vi "DialogCreateClass_HandleTemplatesDialog.vi"(8 "error in (no error)":errorcluster, 10 "AllTemplatesForThisProvider/InheritanceType(Base/Sub)":T1[](array[typedef]), 11 "ClassWriter in":refnum<class "ClassWriter.lvclass">) -> (0 "error out":errorcluster, 2 "TemplatesOut":T1[](array[typedef]), 3 "RefreshClassTemplates":bool)   [LabVIEW 2020, in "ClassWriterNative.lvclass"]
uses:
  <resource>/Framework/Providers/Open_GDS/ClassProviders/Provider_LvNativeClass/ClassWriterNative_class/ClassWriterNative.lvclass
  <resource>/Framework/Providers/Open_GDS/ClassProviders/Provider_BaseClassInterface/ClassTemplateType.ctl
  <resource>/Framework/Providers/Open_GDS/ClassProviders/Provider_BaseClassInterface/ClassWriter_class/ClassWriter.lvclass
  <vilib>/Utility/config.llb/Write Key (String).vi
  <resource>/Framework/Providers/Open_GDS/ClassProviders/Provider_LvNativeClass/ClassWriterNative_class/ClassWriterNative.lvclass/ClassWriterNative.ctl
  <vilib>/Utility/config.llb/NI_LVConfig.lvlib
panel:
  in  "RemoveTemplate":bool
  in  "AddTemplate":bool
  in  "Cancel":bool
  in  "Save":bool
  in  "Down":bool
  in  "Up":bool
  in  "ClassTemplates":i32(listbox) caption="Class Templates"
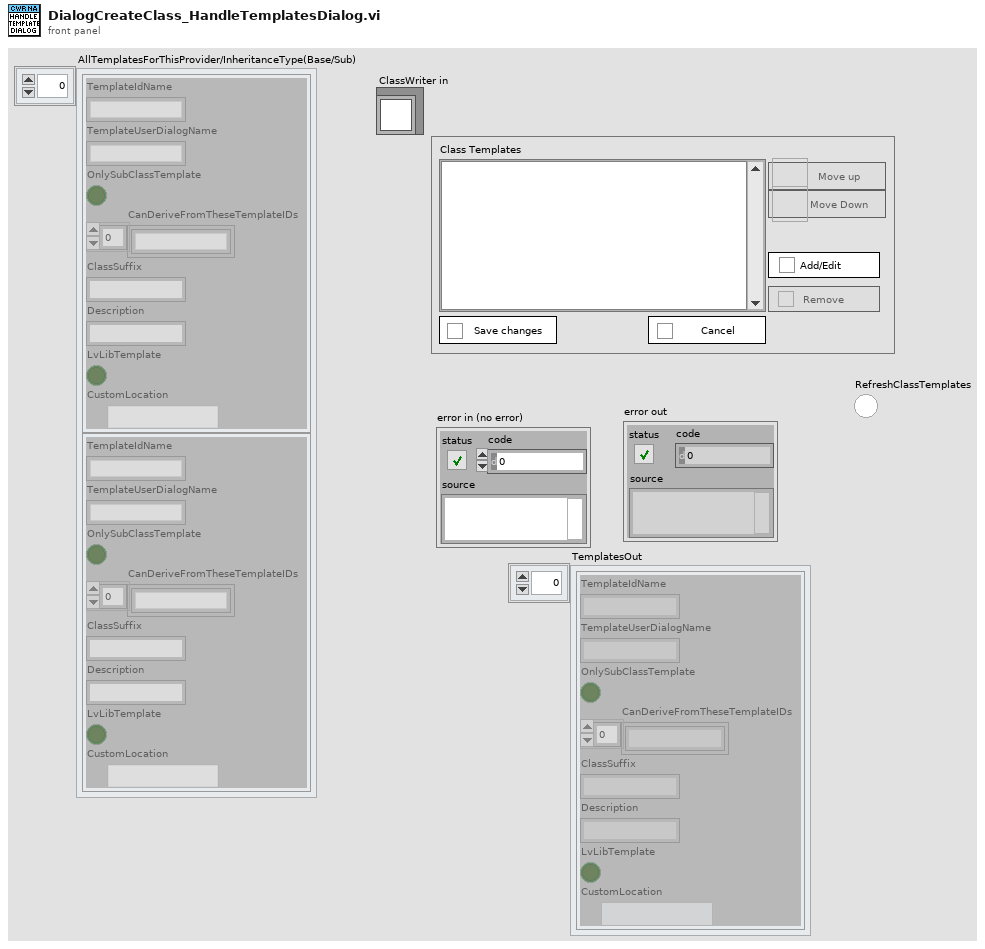
[diagram p1: front panel]
types:
  T1 = typedef "ClassWriter.lvclass/ClassTemplateType.ctl" = cluster{"TemplateIdName":string, "TemplateUserDialogName":string, "OnlySubClassTemplate":bool, "CanDeriveFromTheseTemplateIDs":string[], "ClassSuffix":string, "Description":string, "LvLibTemplate":bool, "CustomLocation":path}
  T2 = cluster{"Section":string, "TemplateIndexSelected":i32, "Templates":T1[], "RefreshClassTemplates":bool, "ProviderShortName":string, "TemplateFilter":cluster{"TemplateNamesSortOrder":string[], "HiddenTemplateNames":string[]}}
  T3 = enum8{"Enabled", "Disabled", "Disabled and Grayed Out"}
  T4 = cluster{"TemplateNamesSortOrder":string[], "HiddenTemplateNames":string[]}
  T5 = cluster{u32, "TemplateUserDialogName":string, bool}
  T6 = cluster{u32, "TemplateUserDialogName":string, bool}[]
  T7 = typedef "LVPoint32TypeDef.ctl" = cluster{"Horizontal":i32, "Vertical":i32}
  T8 = typedef "NI_LVConfig.lvlib/Config Data RefNum.ctl" = refnum<k1>
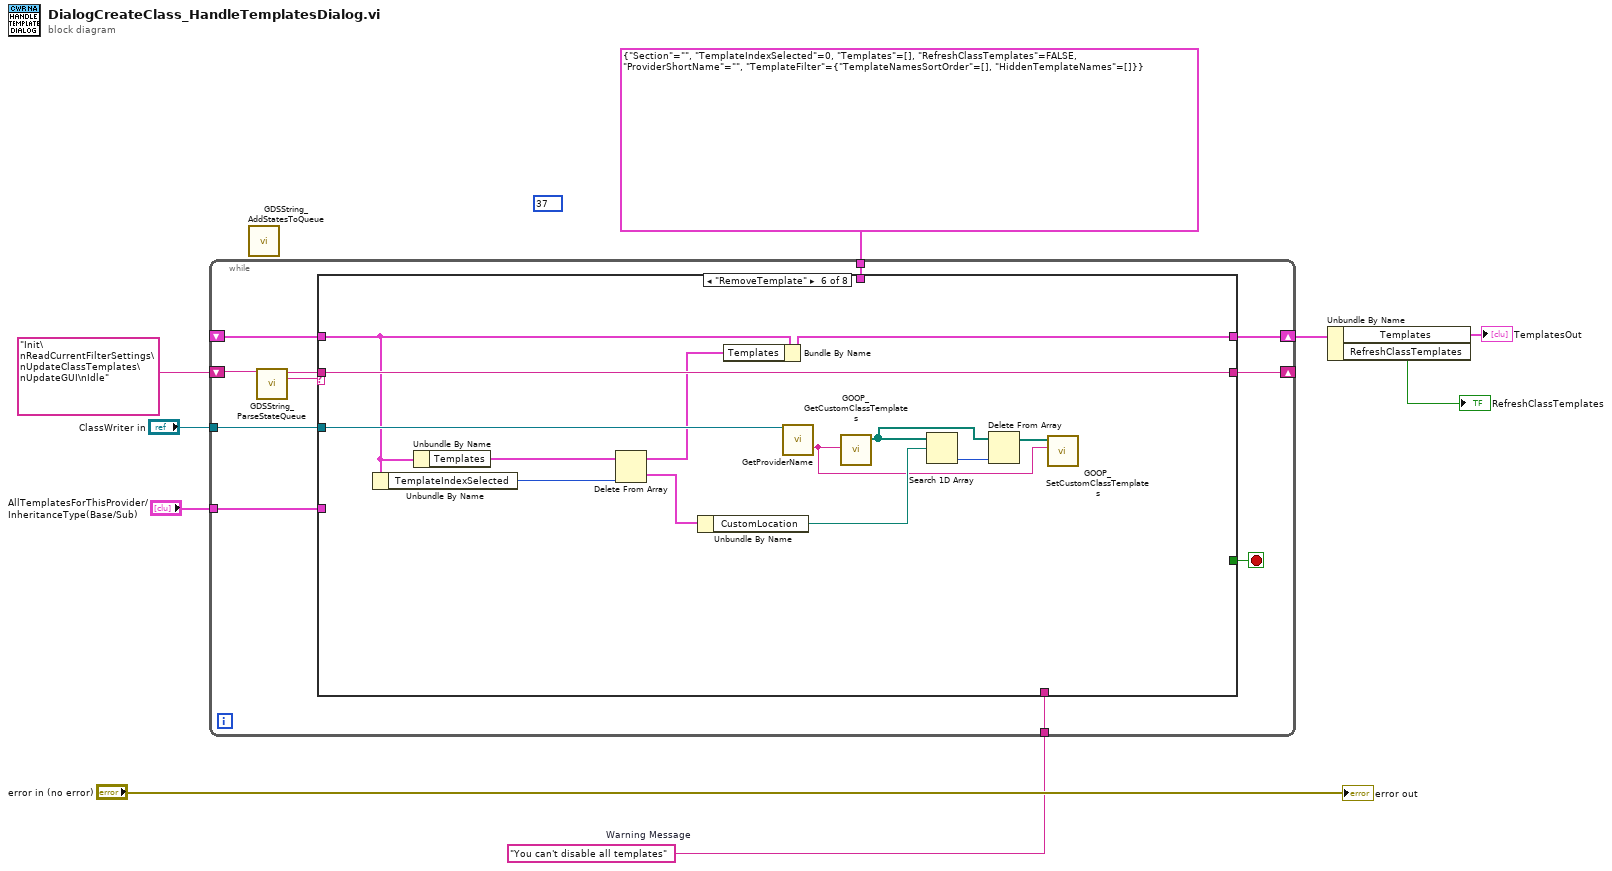
[diagram p0: block diagram]
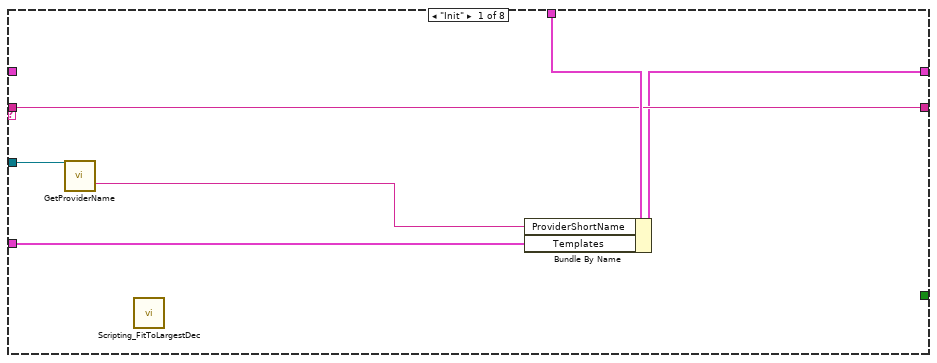
[diagram p2: hidden frame]
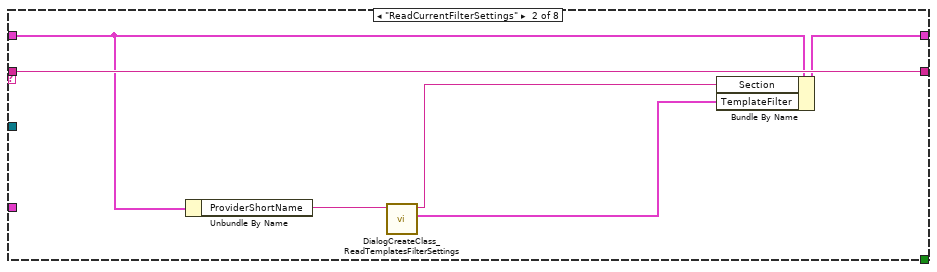
[diagram p3: hidden frame]
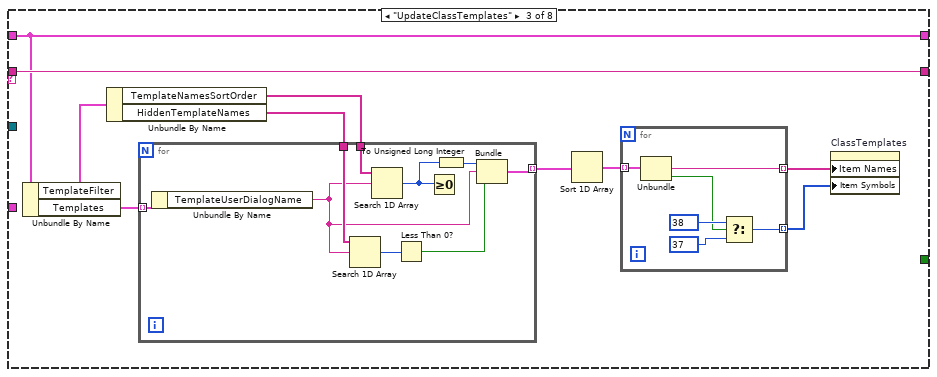
[diagram p4: hidden frame]
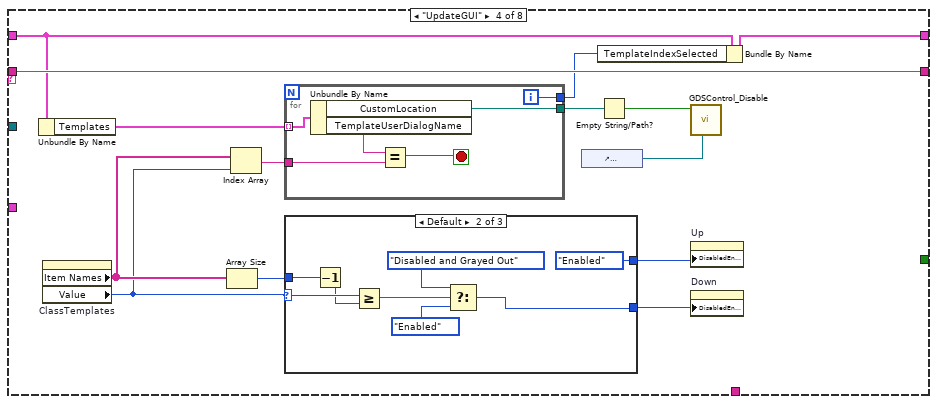
[diagram p5: hidden frame]
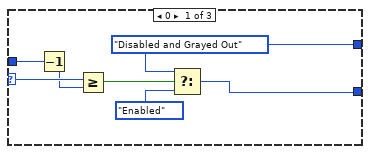
[diagram p6: hidden frame]
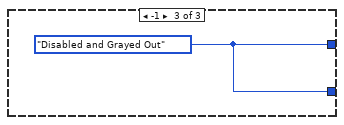
[diagram p7: hidden frame]
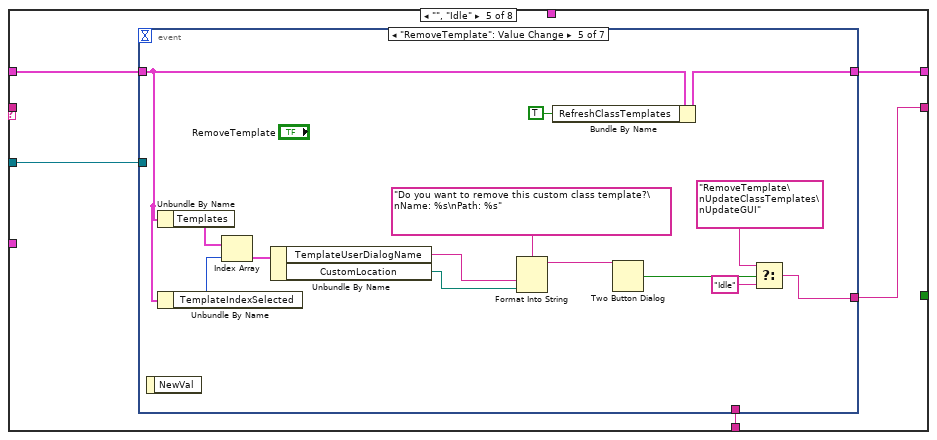
[diagram p8: hidden frame]
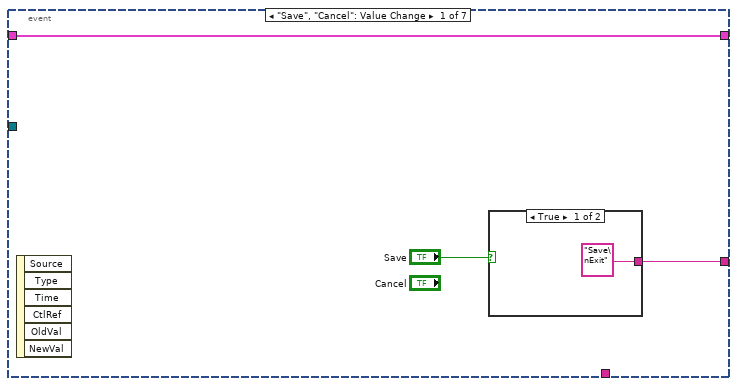
[diagram p9: hidden frame]
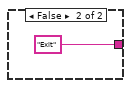
[diagram p10: hidden frame]
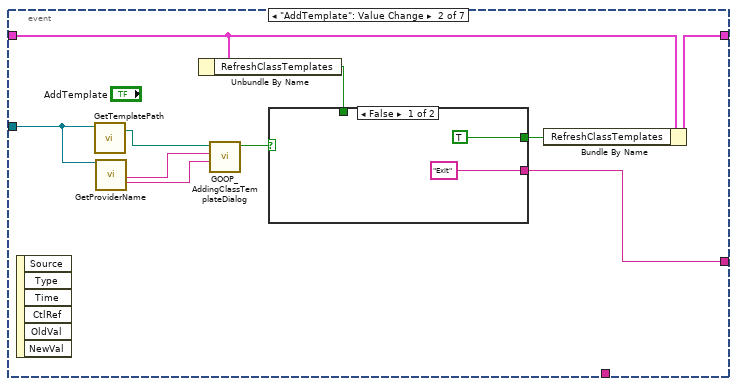
[diagram p11: hidden frame]
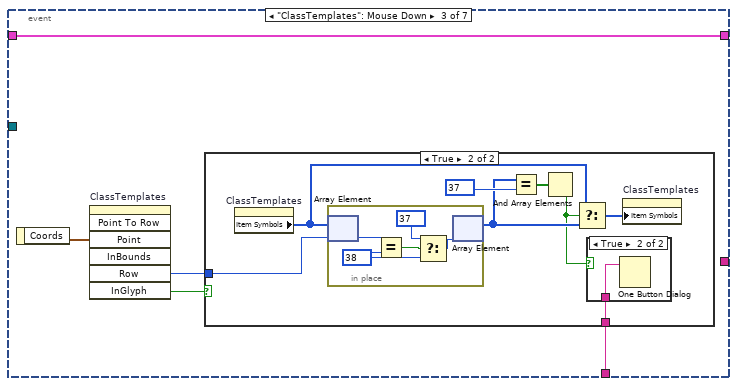
[diagram p13: hidden frame]
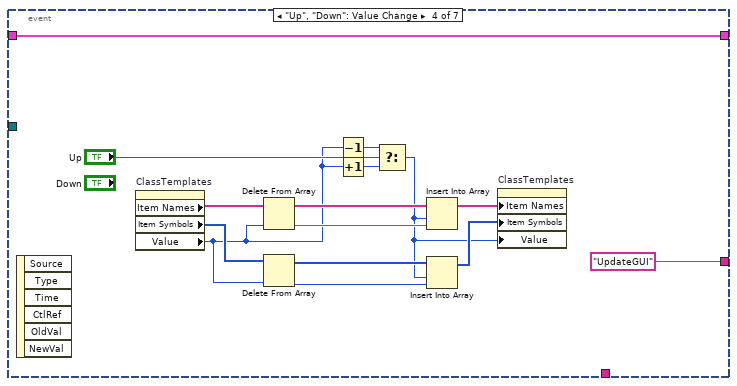
[diagram p16: hidden frame]
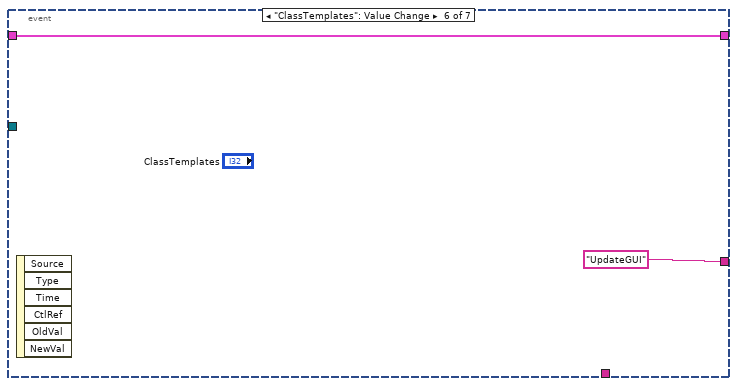
[diagram p17: hidden frame]
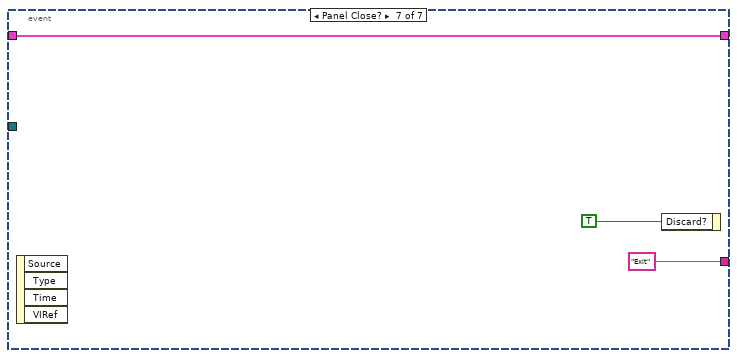
[diagram p18: hidden frame]
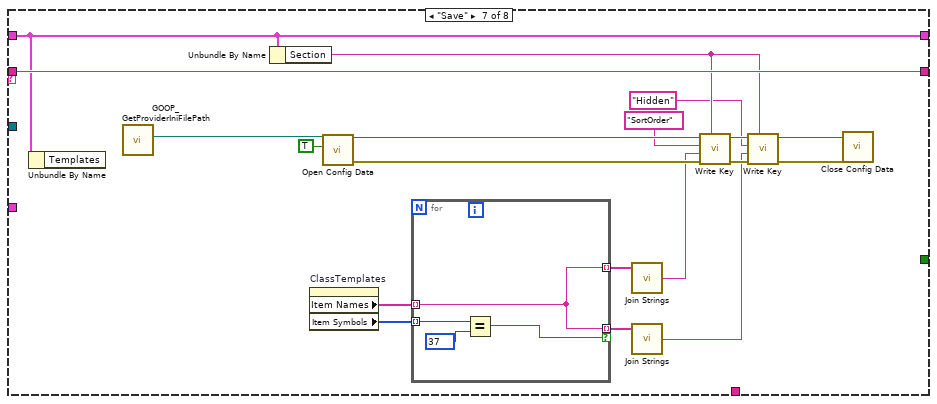
[diagram p19: hidden frame]
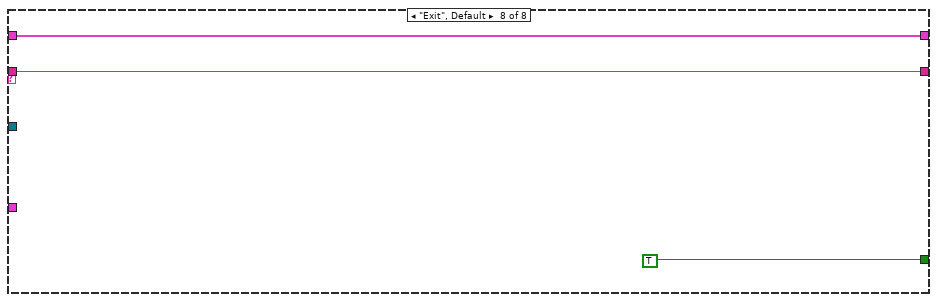
[diagram p20: hidden frame]
diagram:
  (unwired) 37
  w6 = "You can't disable all templates"  # Warning Message
  n1 = while {
    shift-right: [w18] -> _
    shift-left: "Init\nReadCurrentFilterSettings\nUpdateClassTemplates\nUpdateGUI\nIdle" ("Remaining States") -> [w19]
    tunnel: "AllTemplatesForThisProvider/InheritanceType(Base/Sub)" -> [w15]
    tunnel: T2 {"Section"="", "TemplateIndexSelected"=0, "Templates"=[], "RefreshClassTemplates"=FALSE, "ProviderShortName"="", "TemplateFilter"={"TemplateNamesSortOrder"=[], "HiddenTemplateNames"=[]}} -> [w14]
    shift-right: [w13] -> w3
    shift-left: _ -> [w12]
    tunnel: w6 -> [w11]
    tunnel: "ClassWriter in" -> [w10]
    stop <- w20 stop-if-true
    n2 = call <resource>:"GDSString_ParseStateQueue.vi"("State Queue"=w19) -> ("Remaining States"=w16:string, "Current State"=w17:string)  [unwired: 10 in, 3 out]
    n3 = case shown="\"RemoveTemplate\"" w17 {
      tunnel: [_ _ _ _ _ _ _ TRUE] -> w20
      tunnel: [w25 w32 w42 w71 w98 w182 w201 w207] -> w18
      tunnel: w16 -> [w25 w32 w42 w71 _ w182 w201 w207]
      tunnel: w15 -> [w23 _ _ _ _ _ _ _]
      tunnel: [w24 w30 w41 w61 w94 w172 w196 w206] -> w13
      tunnel: w14 -> [w26 _ _ _ _ _ _ _]
      tunnel: w12 -> [_ w28 w41 w59 w96 w176 w196 w206]
      tunnel: w11 -> [_ _ _ _ w97 _ _ _]
      tunnel: w10 -> [w22 _ _ _ w95 w181 _ _]
      frame "Init" {
        n4 = call-dynamic "GetProviderName.vi"("ClassWriter in"=w22) -> ("ShortName(Could be used in for INI Sections)"=w21:string)  [unwired: 14 in, 4 out]
        n5 = call <resource>:"Scripting_FitToLargestDec.vi"() -> ()  [unwired: 6 in, 2 out]
        n6 = Bundle By Name(cluster=w26, "ProviderShortName"=w21, "Templates"=w23) -> (w24:T2)
      }
      frame "ReadCurrentFilterSettings" {
        n7 = Unbundle By Name(w28) -> ("ProviderShortName"=w27:string)
        n8 = call <resource>:"DialogCreateClass_ReadTemplatesFilterSettings.vi"("ProviderShortName"=w27) -> ("TemplateFilter"=w31:T4, "Section"=w29:string)  [unwired: 9 in]
        n9 = Bundle By Name(cluster=w28, "Section"=w29, "TemplateFilter"=w31) -> (w30:T2)
      }
      frame "UpdateClassTemplates" {
        n10 = Unbundle By Name(w41) -> ("TemplateFilter"=w39:T4, "Templates"=w40:T1[])
        n11 = Unbundle By Name(w39) -> ("TemplateNamesSortOrder"=w38:string[], "HiddenTemplateNames"=w35:string[])
        n12 = for {
          tunnel: w40 -> [w57] mode=indexing
          tunnel: w38 -> [w56]
          tunnel: [w53] -> w37 mode=indexing
          tunnel: w35 -> [w52]
          n13 = Unbundle By Name(w57) -> ("TemplateUserDialogName"=w49:string)
          n14 = Search 1D Array(1D array=w52, element=w49) -> (index of element=w51:i32)  [unwired: 1 in]
          n15 = Search 1D Array(1D array=w56, element=w49) -> (index of element=w55:i32)  [unwired: 1 in]
          n16 = Less Than 0?(x=w51) -> (x < 0?=w50:bool)
          n17 = Greater Or Equal To 0?(x=w55) -> ()  [unwired: 1 out]
          n18 = To Unsigned Long Integer(number=w55) -> (unsigned 32bit integer=w54:u32)
          n19 = Bundle(w54, "TemplateUserDialogName"=w49, w50) -> (w53:T5)  [unwired: 1 in]
        }
        n20 = Sort 1D Array(array=w37) -> (sorted array=w36:T6)
        n21 = for {
          tunnel: w36 -> [w48] mode=indexing
          tunnel: [w45] -> w34 mode=indexing
          tunnel: [w44] -> w33 mode=indexing
          n22 = Unbundle(w48) -> ("TemplateUserDialogName"=w45:string, w43:bool)  [unwired: 1 out]
          n23 = Select(t=38, s=w43, f=37) -> (s? t:f=w44:i32)
        }
        n24 = property on="ClassTemplates" class="LstBox (strict)"("Item Names"=w34, "Item Symbols"=w33) -> ()  [unwired: 2 in, 2 out]
      }
      frame "UpdateGUI" {
        n25 = Unbundle By Name(w59) -> ("Templates"=w58:T1[])
        n26 = property on="ClassTemplates" class="LstBox (strict)"() -> ("Item Names"=w67:string[], "Value"=w66:i32)  [unwired: 2 in, 2 out]
        n27 = Array Size(array=w67) -> (size(s)=w68:i32)
        n28 = Index Array(array=w67, index=w66) -> (element=w65:string)
        n29 = for {
          tunnel: w58 -> [w77] mode=indexing
          tunnel: w65 -> [w75]
          tunnel: [w73] -> w64
          tunnel: [w72] -> w60
          i -> [w72]
          stop <- w74 stop-if-true
          n30 = Unbundle By Name(w77) -> ("CustomLocation"=w73:path, "TemplateUserDialogName"=w76:string)
          n31 = Equal?(x=w76, y=w75) -> (x = y?=w74:bool)
        }
        n32 = case shown="Default" w66 {
          selector: w66 -> [w84 w92 _]
          tunnel: [w79 T3."Enabled" ("Disabled") w93] -> w70
          tunnel: [w80 w88 w93] -> w69
          tunnel: w68 -> [w83 w91 _]
          frame 0 {
            w79 = T3."Disabled and Grayed Out" ("Disabled")
            n33 = Decrement(x=w83) -> (x-1=w82:i32)
            n34 = Greater Or Equal?(x=w84, y=w82) -> (x >= y?=w81:bool)
            n35 = Select(t=w79, s=w81, f=T3."Enabled" ("Disabled")) -> (s? t:f=w80:T3)
          }
          frame Default {
            n36 = Decrement(x=w91) -> (x-1=w90:i32)
            n37 = Greater Or Equal?(x=w92, y=w90) -> (x >= y?=w89:bool)
            n38 = Select(t=T3."Disabled and Grayed Out" ("Disabled"), s=w89, f=T3."Enabled" ("Disabled")) -> (s? t:f=w88:T3)
          }
          frame -1 {
            w93 = T3."Disabled and Grayed Out" ("Disabled")
          }
        }
        n39 = control-ref of="RemoveTemplate"() -> (w62:refnum<vi>)
        n40 = Bundle By Name(cluster=w59, "TemplateIndexSelected"=w60) -> (w61:T2)
        n41 = Empty String/Path?(string/path=w64) -> (empty?=w63:bool)
        n42 = call <resource>:"GDSControl_Disable.vi"("ControlRefnum(IgnoreIfNotWired)"=w62, "Disasble(True)"=w63) -> ()  [unwired: 9 in, 1 out]
        n43 = property on="Up" class="Bool"("DisabledEnum"=w70) -> ()  [unwired: 2 in, 2 out]
        n44 = property on="Down" class="Bool"("DisabledEnum"=w69) -> ()  [unwired: 2 in, 2 out]
      }
      frame "", "Idle" {
        n45 = event shown="[4] \"RemoveTemplate\": Value Change" {
          selector: _ -> [_ _ _ _ _ _ _]
          dyn-events: _ -> [_ _ _ _ _ _ _]
          timeout: _ -> [_ _ _ _ _ _ _]
          tunnel: [w101 w108 _ "UpdateGUI" w157 "UpdateGUI" "Exit"] -> w98
          tunnel: w97 -> [_ _ w118 _ _ _ _]
          tunnel: w96 -> [w99 w105 w117 w136 w152 w165 w167]
          tunnel: w95 -> [_ w113 _ _ _ _ _]
          tunnel: [w99 w107 w117 w136 w153 w165 w167] -> w94
          event "Save", "Cancel": Value Change {
            n46 = event-data() -> ()  [unwired: 1 in, 6 out]
            n47 = case shown="True" "Save" {
              tunnel: ["Save\nExit" "Exit"] -> w101
              frame True {
              }
              frame False {
              }
            }
          }
          event "AddTemplate": Value Change {
            n48 = event-data() -> ()  [unwired: 1 in, 6 out]
            n49 = call-dynamic "GetTemplatePath.vi"("ClassWriterIn"=w113) -> ("FolderPathOut"=w112:path)  [unwired: 14 in, 4 out]
            n50 = call-dynamic "GetProviderName.vi"("ClassWriter in"=w113) -> ("TranslatedProviderName"=w111:string, "ShortName(Could be used in for INI Sections)"=w110:string)  [unwired: 14 in, 3 out]
            n51 = Unbundle By Name(w105) -> ("RefreshClassTemplates"=w104:bool)
            n52 = call <resource>:"GOOP_AddingClassTemplateDialog.vi"("ShortName(Could be used in for INI Sections)"=w110, "TranslatedProviderName"=w111, "FolderPathOut"=w112) -> ("Cancelled"=w109:bool)  [unwired: 8 in]
            n53 = case shown="False" w109 {
              tunnel: ["Exit" _] -> w108
              tunnel: [TRUE w116] -> w106
              tunnel: w104 -> [_ w116]
              frame False {
              }
              frame True {
              }
            }
            n54 = Bundle By Name(cluster=w105, "RefreshClassTemplates"=w106) -> (w107:T2)
          }
          event "ClassTemplates": Mouse Down {
            n55 = event-data() -> ("Coords"=w121:T7)  [unwired: 1 in]
            n56 = invoke on="ClassTemplates" class="LstBox (strict)" method="Point To Row"("Point"=w121) -> ("Row"=w119:i32, "InGlyph"=w120:bool)  [unwired: 6 in, 5 out]
            n57 = case shown="True" w120 {
              tunnel: w119 -> [_ w129]
              tunnel: w118 -> [_ w122]
              frame False {
              }
              frame True {
                n58 = property on="ClassTemplates" class="LstBox (strict)"() -> ("Item Symbols"=w125:i32[])  [unwired: 2 in, 2 out]
                n59 = in-place {
                  w133 = 38
                  n60 = in-place-array #1(w125, w129) -> (w135:i32)
                  n61 = Equal?(x=w135, y=w133) -> (x = y?=w134:bool)
                  n62 = Select(t=37, s=w134, f=w133) -> (s? t:f=w131:i32)
                  n63 = in-place-array #1(w131) -> (w126:i32[])  [unwired: 1 out]
                }
                n64 = Equal?(x=w126, y=37) -> (x = y?=w127:bool[])
                n65 = And Array Elements(Boolean array=w127) -> (logical AND=w123:bool)
                n66 = Select(t=w125, s=w123, f=w126) -> (s? t:f=w124:i32[])
                n67 = case shown="True" w123 {
                  tunnel: w122 -> [_ w130]
                  frame False {
                  }
                  frame True {
                    n68 = One Button Dialog(message=w130) -> ()  [unwired: 1 in, 1 out]
                  }
                }
                n69 = property on="ClassTemplates" class="LstBox (strict)"("Item Symbols"=w124) -> ()  [unwired: 2 in, 2 out]
              }
            }
          }
          event "Up", "Down": Value Change {
            n70 = event-data() -> ()  [unwired: 1 in, 6 out]
            n71 = property on="ClassTemplates" class="LstBox (strict)"() -> ("Item Names"=w149:string[], "Item Symbols"=w148:i32[], "Value"=w139:i32)  [unwired: 2 in, 2 out]
            n72 = Delete From Array(array=w149, index=w139) -> (deleted portion=w145:string, array with subset deleted=w147:string[])  [unwired: 1 in]
            n73 = Delete From Array(array=w148, index=w139) -> (deleted portion=w144:i32, array with subset deleted=w146:i32[])  [unwired: 1 in]
            n74 = Decrement(x=w139) -> (x-1=w138:i32)
            n75 = Increment(x=w139) -> (x+1=w137:i32)
            n76 = Select(t=w138, s="Up", f=w137) -> (s? t:f=w140:i32)
            n77 = Insert Into Array(array=w147, index=w140, new element=w145) -> (w142:string[])
            n78 = Insert Into Array(array=w146, index=w140, new element=w144) -> (w141:i32[])
            n79 = property on="ClassTemplates" class="LstBox (strict)"("Item Names"=w142, "Item Symbols"=w141, "Value"=w140) -> ()  [unwired: 2 in, 2 out]
          }
          event "RemoveTemplate": Value Change {
            n80 = event-data() -> ()  [unwired: 1 in, 1 out]
            n81 = Unbundle By Name(w152) -> ("Templates"=w154:T1[])
            n82 = Unbundle By Name(w152) -> ("TemplateIndexSelected"=w163:i32)
            n83 = Index Array(array=w154, index=w163) -> (element=w162:T1)
            n84 = Unbundle By Name(w162) -> ("TemplateUserDialogName"=w161:string, "CustomLocation"=w160:path)
            n85 = Format Into String(format string="Do you want to remove this custom class template?\nName: %s\nPath: %s", w161, w160) -> (resulting string=w159:string)  [unwired: 2 in, 1 out]
            n86 = Bundle By Name(cluster=w152, "RefreshClassTemplates"=TRUE) -> (w153:T2)
            n87 = Two Button Dialog(message=w159) -> (T button?=w158:bool)  [unwired: 2 in]
            n88 = Select(t="RemoveTemplate\nUpdateClassTemplates\nUpdateGUI", s=w158, f="Idle") -> (s? t:f=w157:string)
          }
          event "ClassTemplates": Value Change {
            n89 = event-data() -> ()  [unwired: 1 in, 6 out]
          }
          event Panel Close? {
            n90 = event-data() -> ()  [unwired: 1 in, 4 out]
            n91 = event-data("Discard?"=TRUE) -> ()  [unwired: 1 in, 1 out]
          }
        }
      }
      frame "RemoveTemplate" {
        n92 = Unbundle By Name(w176) -> ("TemplateIndexSelected"=w173:i32)
        n93 = Unbundle By Name(w176) -> ("Templates"=w175:T1[])
        n94 = Delete From Array(array=w175, index=w173) -> (deleted portion=w174:T1, array with subset deleted=w171:T1[])  [unwired: 1 in]
        n95 = Unbundle By Name(w174) -> ("CustomLocation"=w180:path)
        n96 = Bundle By Name(cluster=w176, "Templates"=w171) -> (w172:T2)
        n97 = call-dynamic "GetProviderName.vi"("ClassWriter in"=w181) -> ("ShortName(Could be used in for INI Sections)"=w177:string)  [unwired: 14 in, 4 out]
        n98 = call <resource>:"GOOP_GetCustomClassTemplates.vi"("ClassType"=w177) -> ("CustomTemplates"=w179:path[])  [unwired: 10 in]
        n99 = Search 1D Array(1D array=w179, element=w180) -> (index of element=w170:i32)  [unwired: 1 in]
        n100 = Delete From Array(array=w179, index=w170) -> (array with subset deleted=w178:path[])  [unwired: 1 in, 1 out]
        n101 = call <resource>:"GOOP_SetCustomClassTemplates.vi"("ClassType"=w177, "CustomTemplates"=w178) -> ()  [unwired: 10 in]
      }
      frame "Save" {
        n102 = Unbundle By Name(w196) -> ()  [unwired: 1 out]
        n103 = call <resource>:"GOOP_GetProviderIniFilePath.vi"() -> ("ProviderIniPath"=w199:path)  [unwired: 10 in, 1 out]
        n104 = Unbundle By Name(w196) -> ("Section"=w189:string)
        n105 = property on="ClassTemplates" class="LstBox (strict)"() -> ("Item Names"=w198:string[], "Item Symbols"=w197:i32[])  [unwired: 2 in, 2 out]
        n106 = call <vilib>:"Open Config Data.vi"("create file if necessary (T)"=TRUE, "configuration file path"=w199) -> ("error out"=w195:errorcluster, "refnum"=w194:T8)  [unwired: 7 in, 1 out]
        n107 = for {
          tunnel: w198 -> [w202] mode=indexing
          tunnel: w197 -> [w205] mode=indexing
          tunnel: [w202] -> w186 mode=indexing
          tunnel: [w202] -> w184 mode=indexing if=w203
          n108 = Equal?(x=w205, y=37) -> (x = y?=w203:bool)
        }
        n109 = call <vilib>:"Join Strings.vi"("Strings In"=w186) -> ("String"=w185:string)  [unwired: 2 in]
        n110 = call <vilib>:"Join Strings.vi"("Strings In"=w184) -> ("String"=w183:string)  [unwired: 2 in]
        n111 = call-poly <vilib>:"Write Key.vi"("section"=w189, "error in (no error)"=w195, "value"=w185, "key"="SortOrder", "refnum"=w194) -> ("error out"=w193:errorcluster, "refnum out"=w192:T8)  [unwired: 4 in, 1 out]
        n112 = call-poly <vilib>:"Write Key.vi"("section"=w189, "error in (no error)"=w193, "value"=w183, "key"="Hidden", "refnum"=w192) -> ("error out"=w191:errorcluster, "refnum out"=w190:T8)  [unwired: 4 in, 1 out]
        n113 = call <vilib>:"Close Config Data.vi"("error in (no error)"=w191, "refnum"=w190) -> ()  [unwired: 8 in, 2 out]
      }
      frame "Exit", Default {
      }
    }
  }
  n114 = call <resource>:"GDSString_AddStatesToQueue.vi"() -> ()  [unwired: 15 in, 1 out]
  n115 = Unbundle By Name(w3) -> ("Templates"=→"TemplatesOut":T1[], "RefreshClassTemplates"=→"RefreshClassTemplates":bool)
  "error out" <- "error in (no error)"
